vi "Read MAX evaluation modified.vi"(7 "元配列":string, 8 "逆前削減配列Max Letter X":string, 11 "順前削減配列 Max L X":string) -> (0 "Later Read":string, 1 "リード方向":enum16{"5’→3'", "3'→5'"}(ring), 2 "最長Right Read値":i32, 3 "Right Read MAX":string, 4 "Right Read":string, 6 "Front Read":string)   [LabVIEW 2018]
panel:
  out "配列終了番号":i32
  out "配列開始番号":i32
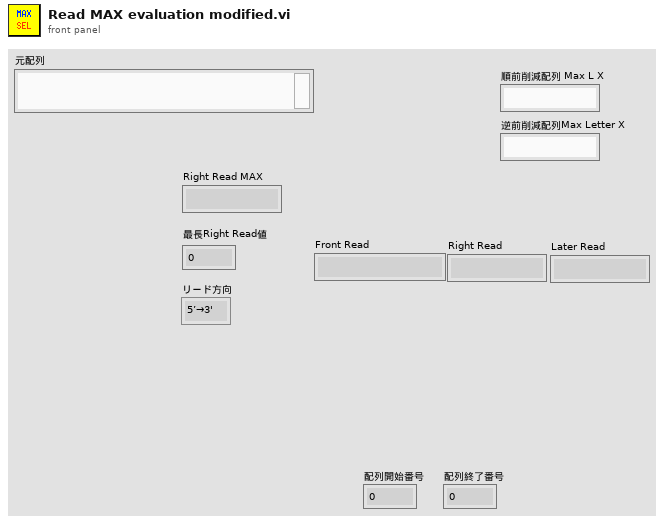
[diagram p1: front panel]
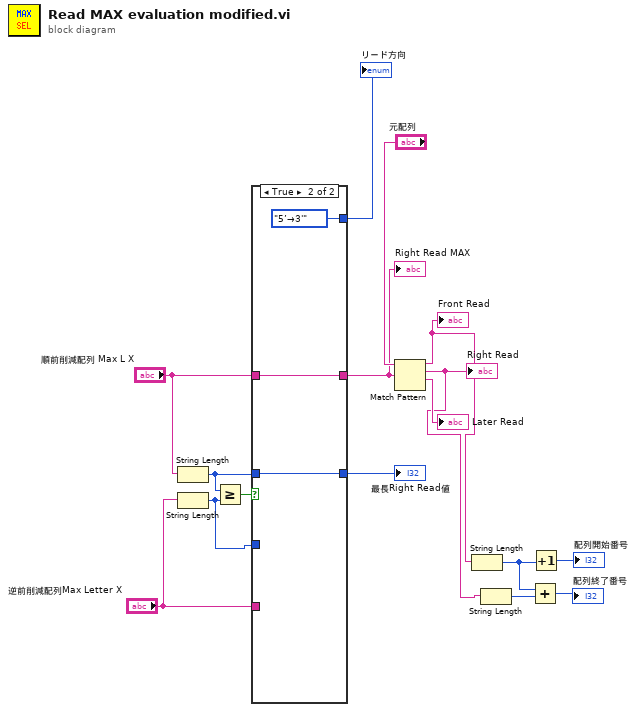
[diagram p0: block diagram]
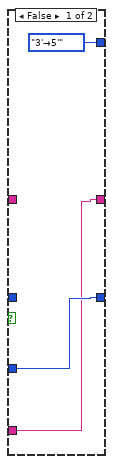
[diagram p2: hidden frame]
diagram:
  n1 = String Length(string="順前削減配列 Max L X") -> (length=w11:i32)
  n2 = String Length(string="逆前削減配列Max Letter X") -> (length=w8:i32)
  n3 = Greater Or Equal?(x=w11, y=w8) -> (x >= y?=w9:bool)
  n4 = case shown="True" w9 {
    tunnel: "順前削減配列 Max L X" -> [_ w22]
    tunnel: w11 -> [_ w21]
    tunnel: [w17 w22] -> w12
    tunnel: [w18 w21] -> w16
    tunnel: [enum16{"5’→3'", "3'→5'"}."3'→5'" ("リード方向") enum16{"5’→3'", "3'→5'"}."5’→3'" ("リード方向")] -> w14
    tunnel: w8 -> [w18 _]
    tunnel: "逆前削減配列Max Letter X" -> [w17 _]
    frame False {
    }
    frame True {
    }
  }
  "Right Read MAX" <- w12
  "最長Right Read値" <- w16
  "リード方向" <- w14
  n5 = Match Pattern(string="元配列", regular expression=w12) -> (before substring=w2:string, match substring=w1:string, after substring=→"Later Read":string)  [unwired: 1 in, 1 out]
  "Front Read" <- w2
  "Right Read" <- w1
  n6 = String Length(string=w2) -> (length=w6:i32)
  n7 = String Length(string=w1) -> (length=w5:i32)
  n8 = Add(x=w6, y=w5) -> (x+y=→"配列終了番号":i32)
  n9 = Increment(x=w6) -> (x+1=→"配列開始番号":i32)
